vi "set TurnTable Parameter.vi"(8 "error in (no error)":errorcluster, 10 "Turn Table Info":T1 {"Target Angle" min=0.0 max=360.0}, 11 "CO3000 in":refnum<class "CO3000.lvclass">) -> (0 "error out":errorcluster, 3 "CO3000 out":refnum<class "CO3000.lvclass">)   [LabVIEW 2023, in "Turn Table and Mast.lvlib" / "CO3000.lvclass"]
uses:
  CO3000.lvclass
  CO3000.lvclass/CO3000.ctl
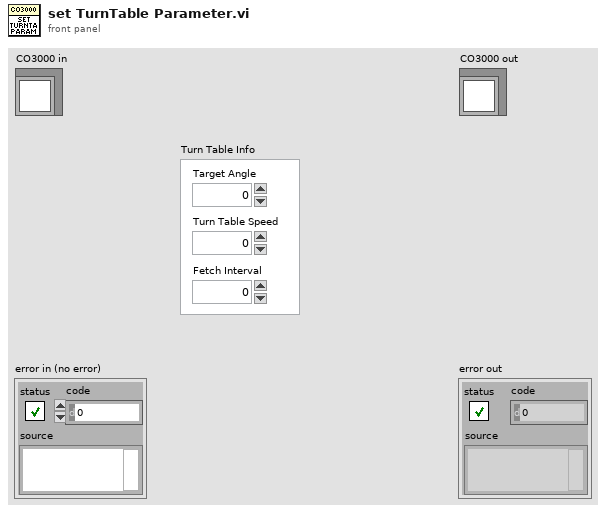
[diagram p1: front panel]
types:
  T1 = cluster{"Target Angle":dbl, "Turn Table Speed":i32, "Fetch Interval":i32}
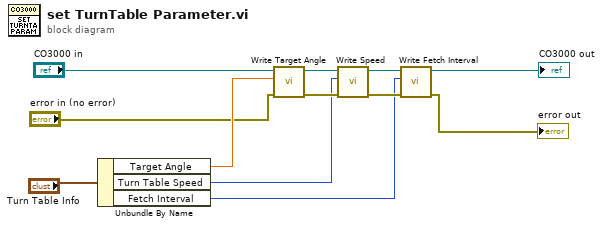
[diagram p0: block diagram]
diagram:
  n1 = Unbundle By Name("Turn Table Info") -> ("Target Angle"=w5:dbl, "Turn Table Speed"=w4:i32, "Fetch Interval"=w3:i32)
  n2 = call "Write Target Angle.vi"("error in (no error)"="error in (no error)", "Target Angle"=w5, "CO3000 in"="CO3000 in") -> ("error out"=w10:errorcluster, "CO3000 out"=w11:refnum<class "CO3000.lvclass">)  [unwired: 7 in]
  n3 = call "Write Speed.vi"("error in (no error)"=w10, "Speed"=w4, "CO3000 in"=w11) -> ("error out"=w8:errorcluster, "CO3000 out"=w9:refnum<class "CO3000.lvclass">)  [unwired: 7 in]
  n4 = call "Write Fetch Interval.vi"("error in (no error)"=w8, "Fetch Interval"=w3, "CO3000 in"=w9) -> ("error out"=→"error out":errorcluster, "CO3000 out"=→"CO3000 out":refnum<class "CO3000.lvclass">)  [unwired: 7 in]
